vi "PicoScope4000aWrapSettings.vi"(9 "Enabled array":i16[](array[numeric]), 10 "Handle In":i16, 11 "error in (no error)":errorcluster) -> (2 "Handle Out":i16, 3 "error out":errorcluster)   [LabVIEW 2009]
uses:
  ps4000aWrap.dll
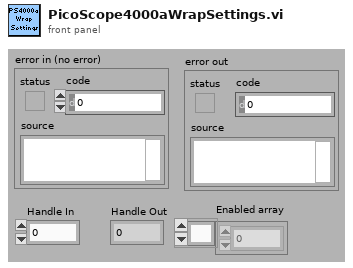
[diagram p1: front panel]
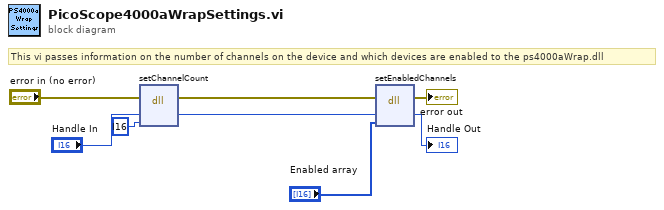
[diagram p0: block diagram]
diagram:
  # "This vi passes information on the number of channels on the device and which devices are enabled to the ps4000aWrap.dll"
  n1 = dll-call lib="ps4000aWrap.dll" fn="setChannelCount"(error in="error in (no error)", "handle"="Handle In", "channelCount"=i16 ?) -> (error out=w3:errorcluster, "handle"=w2:i16)  [unwired: 4 in, 1 out]
  n2 = dll-call lib="ps4000aWrap.dll" fn="setEnabledChannels"(error in=w3, "handle"=w2, "enabledChannels"="Enabled array") -> (error out=→"error out":errorcluster, "handle"=→"Handle Out":i16)  [unwired: 4 in, 1 out]
